vi "Run.vi"(4 "Build Specification Version":T1, 6 "Set PPL Version":bool, 7 "Clear Compiled Object Cache":bool, 8 "error in":errorcluster, 9 "Python Module":path, 10 "Output Folder":path, 11 "Runner in":refnum<class "Runner.lvclass">) -> (0 "error out":errorcluster, 3 "Runner out":refnum<class "Runner.lvclass">)   [LabVIEW 2026, in "Runner.lvlib" / "Runner.lvclass"]
doc: "Run entire generation process through the Runner."
uses:
  Runner.lvclass
  <vilib>/ActorFramework/Actor/Actor.lvclass/Actor.ctl
  <vilib>/ActorFramework/Message Enqueuer/Message Enqueuer.lvclass/Message Enqueuer.ctl
  Interfaces/IRunner/IRunner Messages/Initialize Msg/Initialize Msg.lvclass/Initialize Msg.ctl
  Interfaces/IRunner/IRunner Messages/Prepare Build Specification Msg/Prepare Build Specification Msg.lvclass/Prepare Build Specification Msg.ctl
  Runner.lvclass/Runner.ctl
  C:/Program Files/National Instruments/LabVIEW 2026/vi.lib/ActorFramework/Actor/Actor.lvclass
  C:/Users/juanj/Documents/hasbun_wood_engineering/github/py2vi/labview/Actors/Runner/Runner/Runner.lvclass
  C:/Users/juanj/Documents/hasbun_wood_engineering/github/py2vi/labview/Interfaces/ILogger Client/ILogger Client/ILogger Client.lvclass
  C:/Users/juanj/Documents/hasbun_wood_engineering/github/py2vi/labview/Interfaces/IRunner/IRunner/IRunner.lvclass
  Interfaces/IRunner/IRunner Messages/Initialize Msg/Initialize Msg.lvclass
  Interfaces/IRunner/IRunner Messages/Prepare Project Msg/Prepare Project Msg.lvclass
  Interfaces/IRunner/IRunner Messages/Process Python Code Msg/Process Python Code Msg.lvclass
  Interfaces/IRunner/IRunner Messages/Create Type Definitions Msg/Create Type Definitions Msg.lvclass
  Interfaces/IRunner/IRunner Messages/Create VIs Msg/Create VIs Msg.lvclass
  Interfaces/IRunner/IRunner Messages/Clean Project Msg/Clean Project Msg.lvclass
  <vilib>/ActorFramework/Actor/Actor.lvclass
  <vilib>/ActorFramework/Stop Msg/Stop Msg.lvclass
  Interfaces/IRunner/IRunner Messages/Copy Files Msg/Copy Files Msg.lvclass
  Interfaces/IRunner/IRunner Messages/Populate Type Definitions Msg/Populate Type Definitions Msg.lvclass
  Interfaces/IRunner/IRunner Messages/Populate VIs Msg/Populate VIs Msg.lvclass
  Interfaces/IRunner/IRunner Messages/Add Files to Project Msg/Add Files to Project Msg.lvclass
  Interfaces/IRunner/IRunner Messages/Lint VIs Msg/Lint VIs Msg.lvclass
  Interfaces/IRunner/IRunner Messages/Prepare Build Specification Msg/Prepare Build Specification Msg.lvclass
  <vilib>/AppBuilder/AB_API_Simple/Build Specification Version.ctl
  <vilib>/AppBuilder/AB_API_Simple/NI_App_Builder_API.lvlib
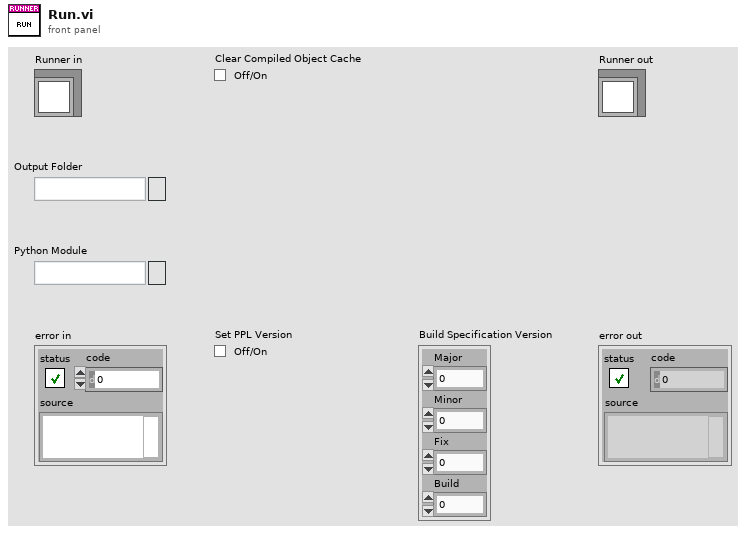
[diagram p1: front panel]
types:
  T1 = typedef "NI_App_Builder_API.lvlib/Build Specification Version.ctl" = cluster{"Major":u16, "Minor":u16, "Fix":u16, "Build":u16}
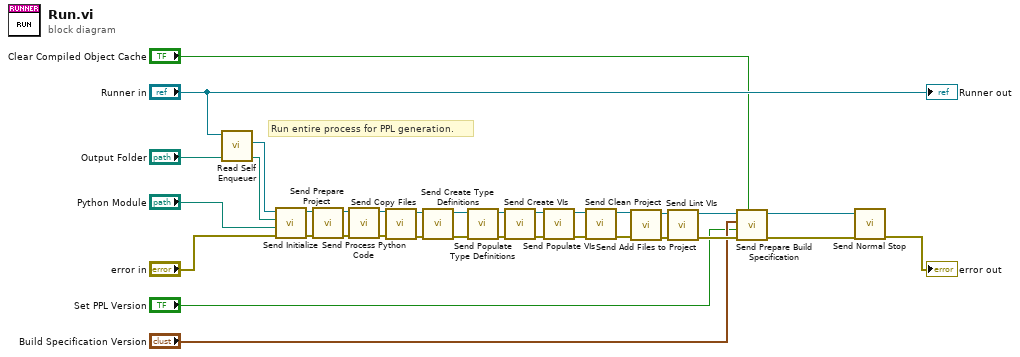
[diagram p0: block diagram]
diagram:
  # "Run entire process for PPL generation."
  n1 = call <vilib>:"Read Self Enqueuer.vi"("Actor"="Runner in") -> ("Self Enqueuer"=w17:refnum<class "Message Enqueuer.lvclass">)  [unwired: 10 in]
  n2 = call "Send Initialize.vi"("error in (no error)"="error in", "Python Module"="Python Module", "Output Folder"="Output Folder", "Message Enqueuer"=w17) -> ("error out"=w32:errorcluster, "Message Enqueuer out"=w18:refnum<class "Message Enqueuer.lvclass">)  [unwired: 6 in]
  n3 = call "Send Prepare Project.vi"("error in (no error)"=w32, "Message Enqueuer"=w18) -> ("error out"=w30:errorcluster, "Message Enqueuer out"=w14:refnum<class "Message Enqueuer.lvclass">)  [unwired: 8 in]
  n4 = call "Send Process Python Code.vi"("error in (no error)"=w30, "Message Enqueuer"=w14) -> ("error out"=w29:errorcluster, "Message Enqueuer out"=w13:refnum<class "Message Enqueuer.lvclass">)  [unwired: 8 in]
  n5 = call "Send Copy Files.vi"("error in (no error)"=w29, "Message Enqueuer"=w13) -> ("error out"=w28:errorcluster, "Message Enqueuer out"=w12:refnum<class "Message Enqueuer.lvclass">)  [unwired: 8 in]
  n6 = call "Send Create Type Definitions.vi"("error in (no error)"=w28, "Message Enqueuer"=w12) -> ("error out"=w27:errorcluster, "Message Enqueuer out"=w11:refnum<class "Message Enqueuer.lvclass">)  [unwired: 8 in]
  n7 = call "Send Populate Type Definitions.vi"("error in (no error)"=w27, "Message Enqueuer"=w11) -> ("error out"=w25:errorcluster, "Message Enqueuer out"=w9:refnum<class "Message Enqueuer.lvclass">)  [unwired: 8 in]
  n8 = call "Send Create VIs.vi"("error in (no error)"=w25, "Message Enqueuer"=w9) -> ("error out"=w26:errorcluster, "Message Enqueuer out"=w10:refnum<class "Message Enqueuer.lvclass">)  [unwired: 8 in]
  n9 = call "Send Populate VIs.vi"("error in (no error)"=w26, "Message Enqueuer"=w10) -> ("error out"=w24:errorcluster, "Message Enqueuer out"=w8:refnum<class "Message Enqueuer.lvclass">)  [unwired: 8 in]
  n10 = call "Send Clean Project.vi"("error in (no error)"=w24, "Message Enqueuer"=w8) -> ("error out"=w23:errorcluster, "Message Enqueuer out"=w7:refnum<class "Message Enqueuer.lvclass">)  [unwired: 8 in]
  n11 = call "Send Add Files to Project.vi"("error in (no error)"=w23, "Message Enqueuer"=w7) -> ("error out"=w22:errorcluster, "Message Enqueuer out"=w6:refnum<class "Message Enqueuer.lvclass">)  [unwired: 8 in]
  n12 = call "Send Lint VIs.vi"("error in (no error)"=w22, "Message Enqueuer"=w6) -> ("error out"=w21:errorcluster, "Message Enqueuer out"=w5:refnum<class "Message Enqueuer.lvclass">)  [unwired: 8 in]
  n13 = call "Send Prepare Build Specification.vi"("Clear Compiled Object Cache"="Clear Compiled Object Cache", "error in (no error)"=w21, "Set PPL Version"="Set PPL Version", "Build Specification Version"="Build Specification Version", "Message Enqueuer"=w5) -> ("error out"=w20:errorcluster, "Message Enqueuer out"=w3:refnum<class "Message Enqueuer.lvclass">)  [unwired: 5 in]
  n14 = call <vilib>:"Send Normal Stop.vi"("error in (no error)"=w20, "Message Enqueuer"=w3) -> ("error out"=→"error out":errorcluster)  [unwired: 9 in]
  "Runner out" <- "Runner in"
